vi "UpdateSubPanel.vi"(8 "error in (no error)":errorcluster, 11 "Navigator in":refnum<class "Navigator.lvclass">) -> (0 "error out":errorcluster, 3 "Navigator out":refnum<class "Navigator.lvclass">)   [LabVIEW 2024, in "Navigator.lvclass"]
doc: "Launch NavigatableView and insert the VI into the Sub Panel."
uses:
  Navigator.lvclass
  Navigator.lvclass/Navigator.ctl
  NavigatableView/NavigatableView.lvclass
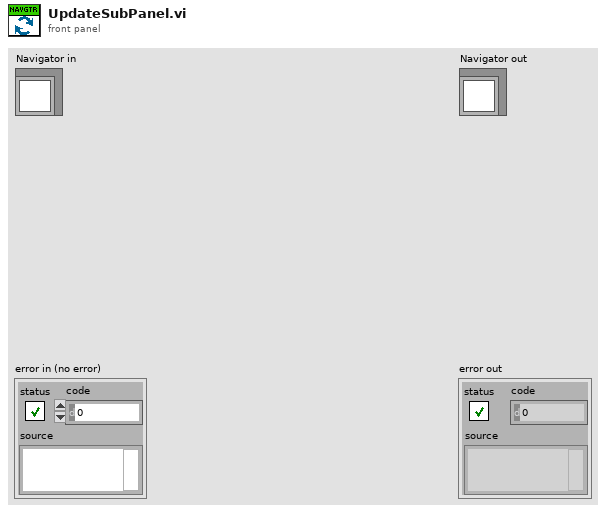
[diagram p1: front panel]
types:
  T1 = typedef "Navigator.lvclass/NavigatorEvents.ctl" = cluster{"go":refnum<user-event>, "push":refnum<user-event>, "pop":refnum<user-event>}
  T2 = typedef "Navigator.lvclass/Route.ctl" = cluster{"Name":string, "Path":path, "Builder":refnum<class "NavigatableView.lvclass">}
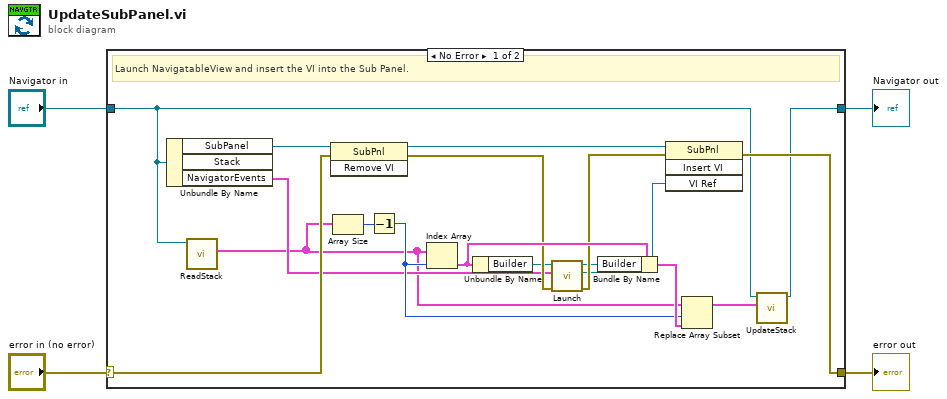
[diagram p0: block diagram]
diagram:
  n1 = case shown="No Error" "error in (no error)" {
    selector: "error in (no error)" -> [w18 w24]
    tunnel: [w19 w24] -> w1
    tunnel: [w5 w23] -> w2
    tunnel: "Navigator in" -> [w7 w23]
    frame No Error {
      # "Launch NavigatableView and insert the VI into the Sub Panel."
      n2 = Unbundle By Name(w7) -> ("SubPanel"=w22:refnum<vi>, "NavigatorEvents"=w10:T1)  [unwired: 1 out]
      n3 = call "ReadStack.vi"("Navigator in"=w7) -> ("Stack"=w8:T2[])  [unwired: 8 in, 2 out]
      n4 = invoke class="SubPnl" method="Remove VI"(reference=w22, error in=w18) -> (reference out=w21:refnum<vi>, error out=w14:errorcluster)  [unwired: 1 in, 1 out]
      n5 = Array Size(array=w8) -> (size(s)=w20:i32)
      n6 = Decrement(x=w20) -> (x-1=w15:i32)
      n7 = Index Array(array=w8, index=w15) -> (element=w17:T2)
      n8 = Unbundle By Name(w17) -> ("Builder"=w11:refnum<class "NavigatableView.lvclass">)
      n9 = call-dynamic "Launch.vi"("error in (no error)"=w14, "NavigatorEvents"=w10, "NavigatableView in"=w11) -> ("error out"=w13:errorcluster, "VIReference"=w9:refnum<vi>, "NavigatableView out"=w12:refnum<class "NavigatableView.lvclass">)  [unwired: 6 in]
      n10 = Bundle By Name(cluster=w17, "Builder"=w12) -> (w16:T2)
      n11 = invoke class="SubPnl" method="Insert VI"(reference=w21, error in=w13, "VI Ref"=w9) -> (error out=w19:errorcluster)  [unwired: 1 in, 3 out]
      n12 = Replace Array Subset(array=w8, new element=w16, index=w15) -> (w6:T2[])
      n13 = call "UpdateStack.vi"("Stack"=w6, "Navigator in"=w7) -> ("Navigator out"=w5:refnum<class "Navigator.lvclass">)  [unwired: 8 in, 1 out]
    }
    frame Error {
    }
  }
  "error out" <- w1
  "Navigator out" <- w2
